vi "iBeam Laser Engine.vi"(0 "iBeam Laser Notifier":string, 11 "COM Port":string[](array[string])) -> ()   [LabVIEW 2016]
uses:
  Laser Controls/Laser Notifier Element.ctl
  Laser Controls/Laser Actions.ctl
  Laser Controls/Laser Settings.ctl
  Laser Controls/Laser Parameters.ctl
  Laser Controls/Laser Status.ctl
  <vilib>/Instr/_visa.llb/VISA Configure Serial Port (Instr).vi
panel:
  in  "Fine A":dbl
  in  "Fine B":dbl
  in  "Enable Fine":bool
  out "Channels":enum32{"Channel 1", "Channel 2"}(radio)
  in  "Get Status":bool
  in  "Get Power":bool
  out "Laser Status":string
  out "Power (uW)":string
  out "Startup Error":errorcluster
  in  "Quit":bool
  in  "Enable Ext":bool
  in  "Laser Power (mW)":dbl
  in  "Laser On/Off":bool
  out "Serial Number":string
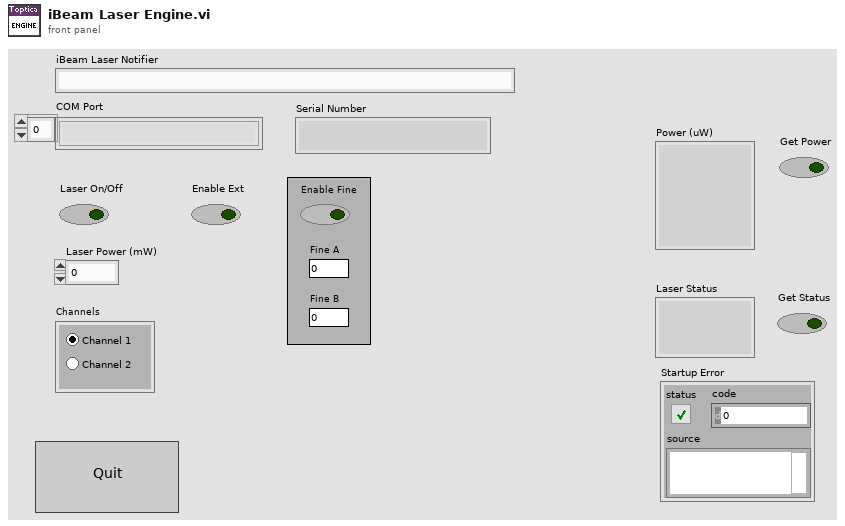
[diagram p1: front panel]
types:
  T1 = typedef "Laser Parameters.ctl" = enum16{"Wavelength (nm)", "Pulsing?", "Rep. Rate", "External Control", "Enable Fine", "Fine A", "Fine B", "Channel No."}
  T2 = typedef "Laser Notifier Element.ctl" = cluster{"Laser Action":T3, "Received?":bool, "Enabled (Interlock)?":bool, "Light Emission?":bool, "Power (mW)":dbl, "Settings":T4, "Status":T5, "Error":errorcluster}
  T3 = typedef "Laser Actions.ctl" = enum16{"Error Check", "Set On/Off", "Set Power", "Set Parameter", "Get Power", "Get Status", "Get Parameter", "Quit"}
  T4 = typedef "Laser Settings.ctl" = cluster{"Laser Parameters":T1, "Value":dbl}
  T5 = typedef "Laser Status.ctl" = enum16{"Warmup", "Ready", "Emission", "Tuning", "Error"}
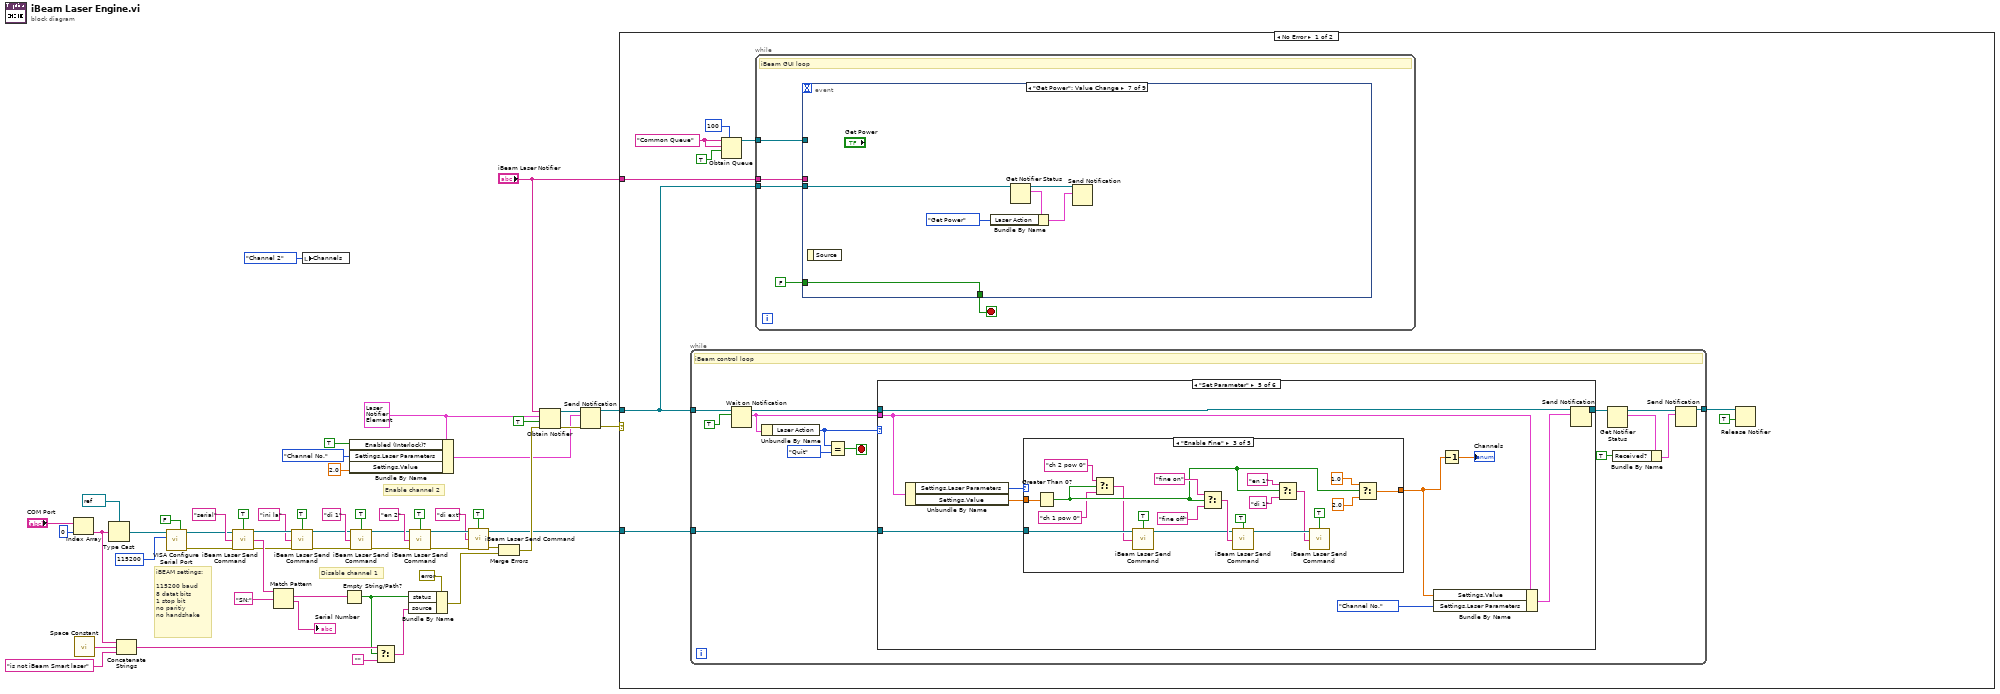
[diagram p0: block diagram]
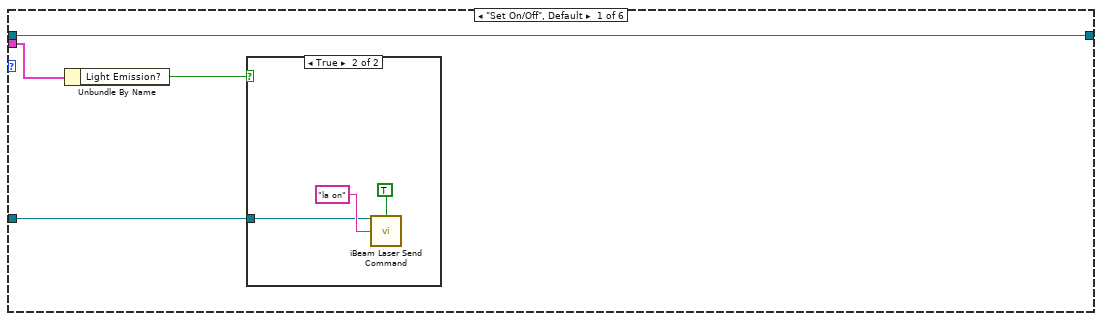
[diagram p2: hidden frame]
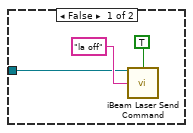
[diagram p3: hidden frame]
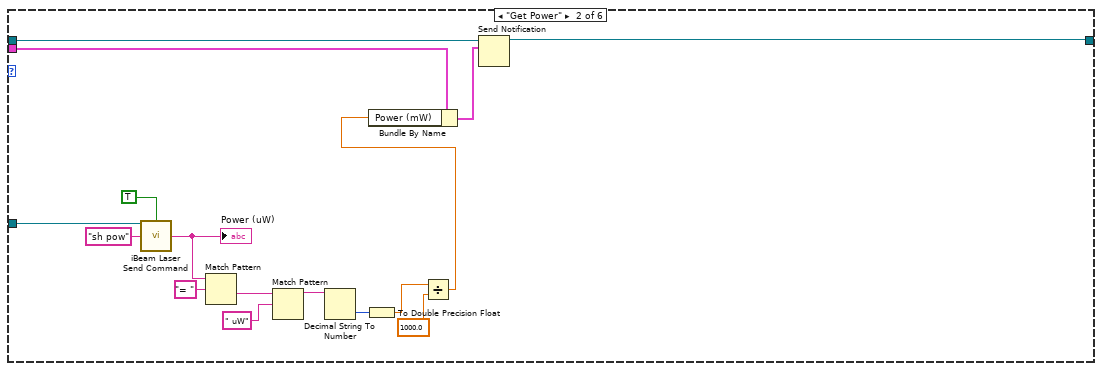
[diagram p4: hidden frame]
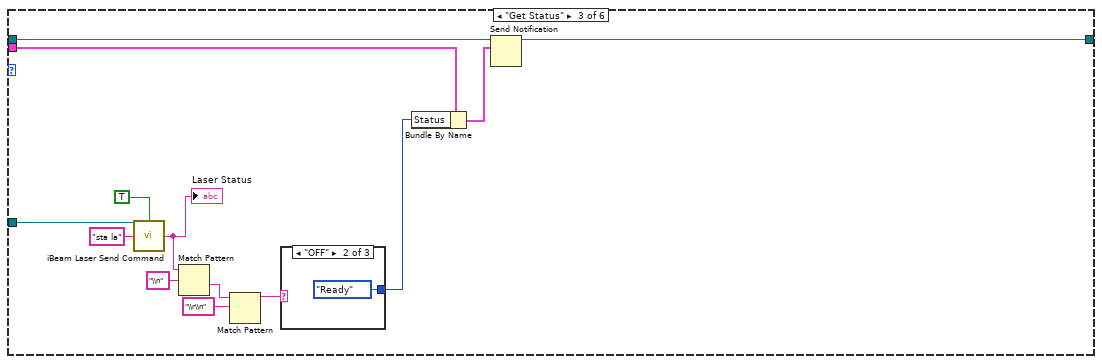
[diagram p5: hidden frame]
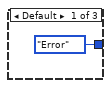
[diagram p6: hidden frame]
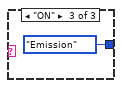
[diagram p7: hidden frame]
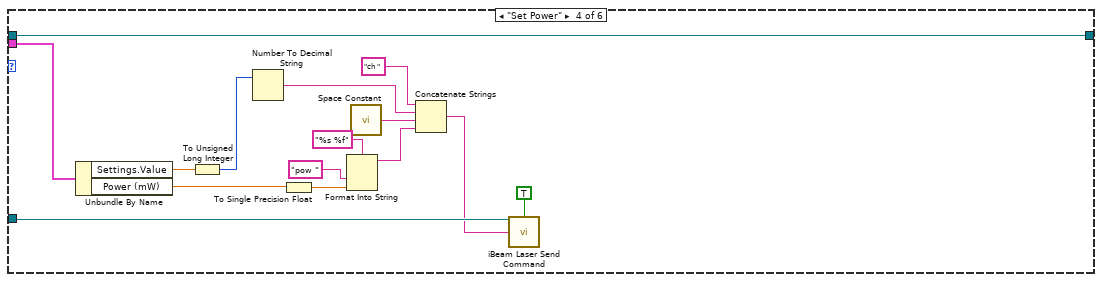
[diagram p8: hidden frame]
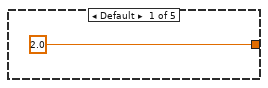
[diagram p9: hidden frame]
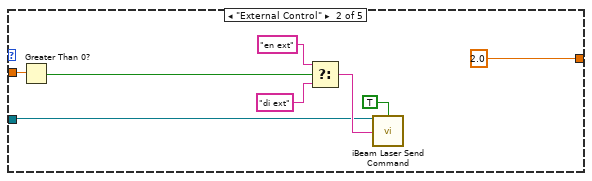
[diagram p10: hidden frame]
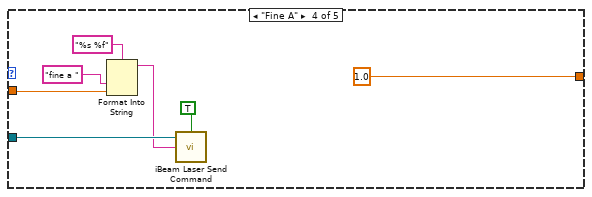
[diagram p11: hidden frame]
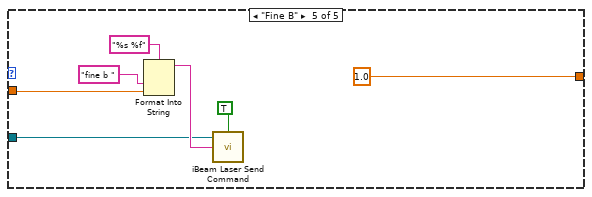
[diagram p12: hidden frame]
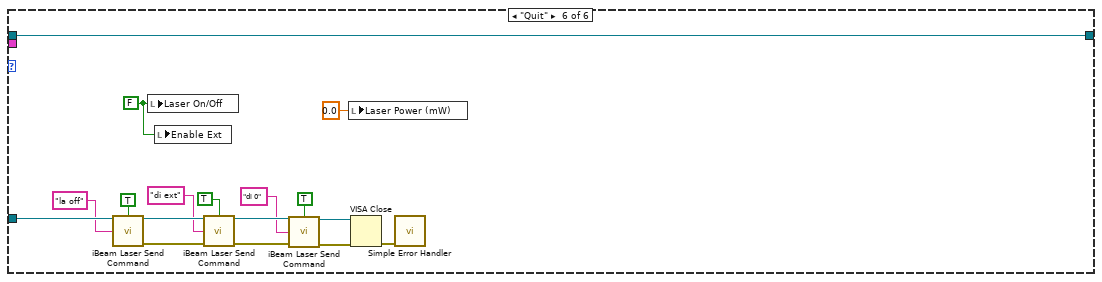
[diagram p13: hidden frame]
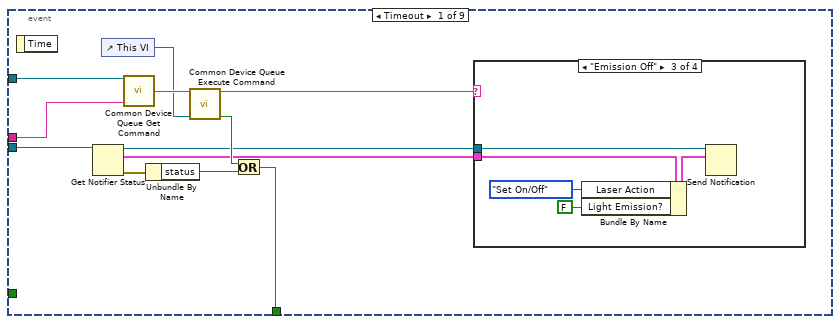
[diagram p14: hidden frame]
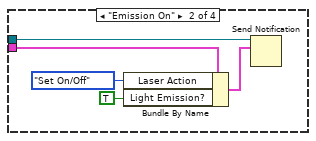
[diagram p16: hidden frame]
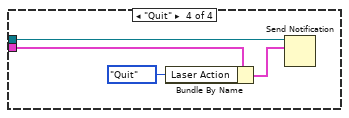
[diagram p17: hidden frame]
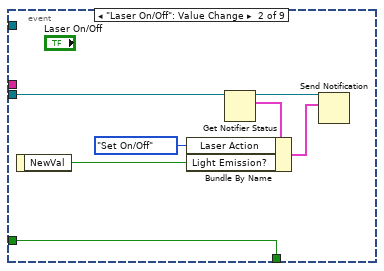
[diagram p18: hidden frame]
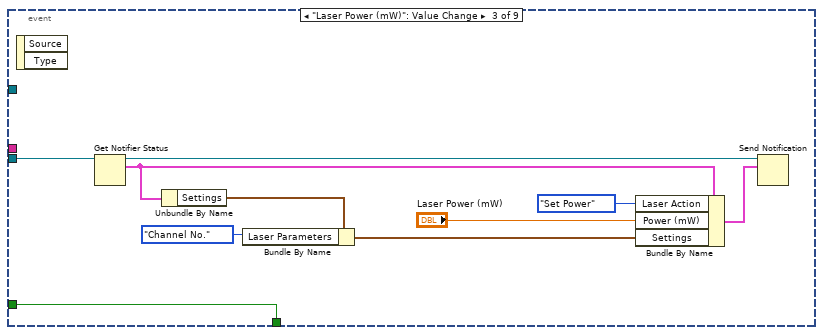
[diagram p19: hidden frame]
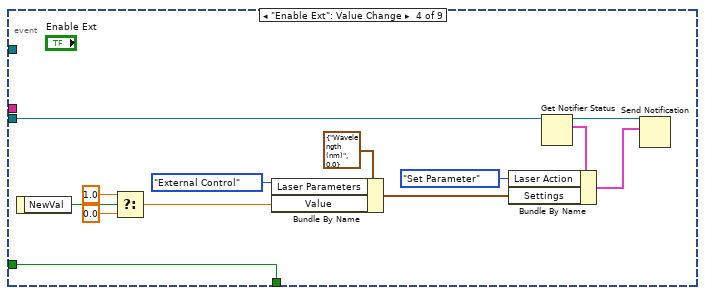
[diagram p20: hidden frame]
diagram:
  w17 = T2 {"Laser Action"=enum."Set On/Off", "Received?"=FALSE, "Enabled (Interlock)?"=FALSE, "Light Emission?"=FALSE, "Power (mW)"=0.0, "Settings"={"Laser Parameters"=enum."Wavelength (nm)", "Value"=0.0}, "Status"=enum."Error", "Error"={"status"=FALSE, "code"=0, "source"=""}} ("Laser Notifier Element")
  # "iBEAM settings:\n\n115200 baud\n8 datat bits\n1 stop bit\nno paritiy\nno handshake"
  # "Enable channel 2"
  # "Disable channel 1"
  n1 = Index Array(array="COM Port", index=0) -> (element=w47:string)
  n2 = call <vilib>:"Space Constant.vi"() -> ("String"=w46:string)
  n3 = Type Cast(type=refnum<visa-resource-name> refnum ("VISA resource name"), x=w47) -> (*(type *) &x=w6:refnum<visa-resource-name>)
  n4 = Concatenate Strings(w47, w46, "is not iBeam Smart laser" ("string")) -> (w43:string)
  n5 = call-poly "VISA Configure Serial Port"("VISA resource name"=w6, "Enable Termination\nChar (T)"=FALSE ("Enable Termination\nChar (T)"), "baud rate (9600)"=u32 115200 ("baud rate (115200)")) -> ("VISA resource name out"=w5:refnum<visa-resource-name>, "error out"=w4:errorcluster)  [unwired: 11 in]
  n6 = call "iBeam Laser Send Command.vi"("VISA Ref"=w5, "Wait for Reply?"=TRUE, "Command"="serial" ("command"), "Error In"=w4) -> ("VISA Ref Out"=w33:refnum<visa-resource-name>, "Response"=w50:string, "Error Out"=w32:errorcluster)  [unwired: 9 in]
  n7 = Match Pattern(string=w50, regular expression="SN:") -> (match substring=w44:string, after substring=→"Serial Number":string)  [unwired: 1 in, 2 out]
  n8 = call "iBeam Laser Send Command.vi"("VISA Ref"=w33, "Wait for Reply?"=TRUE, "Command"="ini la", "Error In"=w32) -> ("VISA Ref Out"=w25:refnum<visa-resource-name>, "Error Out"=w24:errorcluster)  [unwired: 9 in, 1 out]
  n9 = local write "Channels"(enum32{"Channel 1", "Channel 2"}."Channel 2" ("Channels")) -> ()
  n10 = Empty String/Path?(string/path=w44) -> (empty?=w40:bool)
  n11 = Bundle By Name(cluster=w17, "Enabled (Interlock)?"=TRUE, "Settings.Laser Parameters"=Laser_Parameters."Channel No.", "Settings.Value"=2.0) -> (w15:T2)
  n12 = call "iBeam Laser Send Command.vi"("VISA Ref"=w25, "Wait for Reply?"=TRUE, "Command"="di 1", "Error In"=w24) -> ("VISA Ref Out"=w22:refnum<visa-resource-name>, "Error Out"=w21:errorcluster)  [unwired: 9 in, 1 out]
  n13 = Select(t=w43, s=w40, f="") -> (s? t:f=w39:string)
  n14 = Bundle By Name(cluster=errorcluster {"status"=FALSE, "code"=0, "source"=""} ("error in"), "status"=w40, "source"=w39) -> (w38:errorcluster)
  n15 = call "iBeam Laser Send Command.vi"("VISA Ref"=w22, "Wait for Reply?"=TRUE, "Command"="en 2", "Error In"=w21) -> ("VISA Ref Out"=w14:refnum<visa-resource-name>, "Error Out"=w11:errorcluster)  [unwired: 9 in, 1 out]
  n16 = call "iBeam Laser Send Command.vi"("VISA Ref"=w14, "Wait for Reply?"=TRUE, "Command"="di ext", "Error In"=w11) -> ("VISA Ref Out"=w13:refnum<visa-resource-name>, "Error Out"=w10:errorcluster)  [unwired: 9 in, 1 out]
  n17 = Merge Errors(w10, w38) -> (w37:errorcluster)
  n18 = Obtain Notifier(name (unnamed)="iBeam Laser Notifier", notification data type=w17, create if not found? (T)=TRUE, error in (no error)=w37) -> (notifier out=w27:refnum<notifier>, error out=w36:errorcluster)  [unwired: 1 out]
  n19 = Send Notification(notification=w15, notifier=w27, error in (no error)=w36) -> (notifier out=w29:refnum<notifier>, error out=w35:errorcluster)
  n20 = case shown="No Error" w35 {
    selector: w35 -> [_ w310]
    tunnel: w29 -> [w63 w311]
    tunnel: w13 -> [w62 w309]
    tunnel: "iBeam Laser Notifier" -> [w56 _]
    frame No Error {
      w59 = "Common Queue" ("Unique Notifier Name")
      n21 = while {
        tunnel: w63 -> [w77]
        tunnel: w62 -> [w73]
        tunnel: [w65] -> w60
        stop <- w76 stop-if-true
        # "iBeam control loop"
        n22 = Wait on Notification(notifier=w77, ignore previous (F)=TRUE) -> (notifier out=w72:refnum<notifier>, notification=w74:T2)  [unwired: 2 in, 2 out]
        n23 = Unbundle By Name(w74) -> ("Laser Action"=w75:T3)
        n24 = Equal?(x=w75, y=Laser_Actions."Quit") -> (x = y?=w76:bool)
        n25 = case shown="\"Set Parameter\"" w75 {
          tunnel: w74 -> [w81 w92 w108 w134 w140 _]
          tunnel: w73 -> [w79 w103 w116 w129 w144 w204]
          tunnel: w72 -> [w78 w90 w105 w126 w138 w188]
          tunnel: [w78 w89 w104 w126 w139 w188] -> w70
          frame "Set On/Off", Default {
            n26 = Unbundle By Name(w81) -> ("Light Emission?"=w80:bool)
            n27 = case shown="True" w80 {
              tunnel: w79 -> [w82 w85]
              frame False {
                n28 = call "iBeam Laser Send Command.vi"("VISA Ref"=w82, "Wait for Reply?"=TRUE, "Command"="la off" ("command")) -> ()  [unwired: 10 in, 3 out]
              }
              frame True {
                n29 = call "iBeam Laser Send Command.vi"("VISA Ref"=w85, "Wait for Reply?"=TRUE, "Command"="la on" ("command")) -> ()  [unwired: 10 in, 3 out]
              }
            }
          }
          frame "Get Power" {
            n30 = call "iBeam Laser Send Command.vi"("VISA Ref"=w103, "Wait for Reply?"=TRUE, "Command"="sh pow") -> ("Response"=w100:string)  [unwired: 10 in, 2 out]
            "Power (uW)" <- w100
            n31 = Match Pattern(string=w100, regular expression="= ") -> (after substring=w98:string)  [unwired: 1 in, 3 out]
            n32 = Match Pattern(string=w98, regular expression=" uW") -> (before substring=w96:string)  [unwired: 1 in, 3 out]
            n33 = Decimal String To Number(string=w96) -> (number=w95:i32)  [unwired: 2 in, 1 out]
            n34 = To Double Precision Float(number=w95) -> (double precision float=w94:dbl)
            n35 = Divide(x=w94, y=1000.0) -> (x/y=w88:dbl)
            n36 = Bundle By Name(cluster=w92, "Power (mW)"=w88) -> (w91:T2)
            n37 = Send Notification(notification=w91, notifier=w90) -> (notifier out=w89:refnum<notifier>)  [unwired: 1 in, 1 out]
          }
          frame "Get Status" {
            n38 = call "iBeam Laser Send Command.vi"("VISA Ref"=w116, "Wait for Reply?"=TRUE, "Command"="sta la") -> ("Response"=w113:string)  [unwired: 10 in, 2 out]
            "Laser Status" <- w113
            n39 = Match Pattern(string=w113, regular expression="\\n") -> (after substring=w112:string)  [unwired: 1 in, 3 out]
            n40 = Match Pattern(string=w112, regular expression="\\r\\n") -> (before substring=w109:string)  [unwired: 1 in, 3 out]
            n41 = case shown="\"OFF\"" w109 {
              tunnel: [Laser_Status."Error" ("Status") Laser_Status."Ready" ("Status") Laser_Status."Emission" ("Status")] -> w107
              frame Default {
              }
              frame "OFF" {
              }
              frame "ON" {
              }
            }
            n42 = Bundle By Name(cluster=w108, "Status"=w107) -> (w106:T2)
            n43 = Send Notification(notification=w106, notifier=w105) -> (notifier out=w104:refnum<notifier>)  [unwired: 1 in, 1 out]
          }
          frame "Set Power" {
            n44 = Unbundle By Name(w134) -> ("Settings.Value"=w123:dbl, "Power (mW)"=w125:dbl)
            n45 = To Unsigned Long Integer(number=w123) -> (unsigned 32bit integer=w121:u32)
            n46 = Number To Decimal String(number=w121) -> (decimal integer string=w120:string)  [unwired: 1 in]
            n47 = To Single Precision Float(number=w125) -> (single precision float=w124:sgl)
            n48 = Format Into String(format string="%s %f", "pow " ("string"), w124) -> (resulting string=w130:string)  [unwired: 2 in, 1 out]
            n49 = call <vilib>:"Space Constant.vi"() -> ("String"=w131:string)
            n50 = Concatenate Strings("ch " ("string"), w120, w131, w130) -> (w128:string)
            n51 = call "iBeam Laser Send Command.vi"("VISA Ref"=w129, "Wait for Reply?"=TRUE, "Command"=w128) -> ()  [unwired: 10 in, 3 out]
          }
          frame "Set Parameter" {
            n52 = Unbundle By Name(w140) -> ("Settings.Laser Parameters"=w143:T1, "Settings.Value"=w142:dbl)
            n53 = case shown="\"Enable Fine\"" w143 {
              tunnel: w144 -> [_ w146 w159 w176 w182]
              tunnel: w142 -> [_ w152 w169 w178 w183]
              tunnel: [2.0 ("f") 2.0 ("f") w161 1.0 ("f") 1.0 ("f")] -> w136
              frame Default {
              }
              frame "External Control" {
                n54 = Greater Than 0?(x=w152) -> (x > 0?=w148:bool)
                n55 = Select(t="en ext" ("Command"), s=w148, f="di ext" ("Command")) -> (s? t:f=w149:string)
                n56 = call "iBeam Laser Send Command.vi"("VISA Ref"=w146, "Wait for Reply?"=TRUE, "Command"=w149) -> ()  [unwired: 10 in, 3 out]
              }
              frame "Enable Fine" {
                n57 = Greater Than 0?(x=w169) -> (x > 0?=w157:bool)
                n58 = Select(t="ch 2 pow 0" ("Command"), s=w157, f="ch 1 pow 0") -> (s? t:f=w154:string)
                n59 = call "iBeam Laser Send Command.vi"("VISA Ref"=w159, "Wait for Reply?"=TRUE, "Command"=w154) -> ("VISA Ref Out"=w158:refnum<visa-resource-name>)  [unwired: 10 in, 2 out]
                n60 = Select(t="fine on" ("Command"), s=w157, f="fine off" ("Command")) -> (s? t:f=w173:string)
                n61 = call "iBeam Laser Send Command.vi"("VISA Ref"=w158, "Wait for Reply?"=TRUE, "Command"=w173) -> ("VISA Ref Out"=w167:refnum<visa-resource-name>)  [unwired: 10 in, 2 out]
                n62 = Select(t="en 1" ("Command"), s=w157, f="di 1") -> (s? t:f=w164:string)
                n63 = call "iBeam Laser Send Command.vi"("VISA Ref"=w167, "Wait for Reply?"=TRUE, "Command"=w164) -> ()  [unwired: 10 in, 3 out]
                n64 = Select(t=1.0, s=w157, f=2.0) -> (s? t:f=w161:dbl)
              }
              frame "Fine A" {
                n65 = Format Into String(format string="%s %f", "fine a " ("string"), w178) -> (resulting string=w175:string)  [unwired: 2 in, 1 out]
                n66 = call "iBeam Laser Send Command.vi"("VISA Ref"=w176, "Wait for Reply?"=TRUE, "Command"=w175) -> ()  [unwired: 10 in, 3 out]
              }
              frame "Fine B" {
                n67 = Format Into String(format string="%s %f", "fine b " ("string"), w183) -> (resulting string=w187:string)  [unwired: 2 in, 1 out]
                n68 = call "iBeam Laser Send Command.vi"("VISA Ref"=w182, "Wait for Reply?"=TRUE, "Command"=w187) -> ()  [unwired: 10 in, 3 out]
              }
            }
            n69 = Bundle By Name(cluster=w140, "Settings.Value"=w136, "Settings.Laser Parameters"=Laser_Parameters."Channel No." ("Laser Parameters")) -> (w137:T2)
            n70 = Decrement(x=w136) -> (x-1=→"Channels":dbl)
            n71 = Send Notification(notification=w137, notifier=w138) -> (notifier out=w139:refnum<notifier>)  [unwired: 1 in, 1 out]
          }
          frame "Quit" {
            w190 = FALSE ("Laser On/Off")
            n72 = call "iBeam Laser Send Command.vi"("VISA Ref"=w204, "Wait for Reply?"=TRUE, "Command"="la off") -> ("VISA Ref Out"=w202:refnum<visa-resource-name>, "Error Out"=w201:errorcluster)  [unwired: 10 in, 1 out]
            n73 = local write "Laser On/Off"(w190) -> ()
            n74 = local write "Enable Ext"(w190) -> ()
            n75 = call "iBeam Laser Send Command.vi"("VISA Ref"=w202, "Wait for Reply?"=TRUE, "Command"="di ext", "Error In"=w201) -> ("VISA Ref Out"=w196:refnum<visa-resource-name>, "Error Out"=w195:errorcluster)  [unwired: 9 in, 1 out]
            n76 = call "iBeam Laser Send Command.vi"("VISA Ref"=w196, "Wait for Reply?"=TRUE, "Command"="di 0", "Error In"=w195) -> ("VISA Ref Out"=w194:refnum<visa-resource-name>, "Error Out"=w193:errorcluster)  [unwired: 9 in, 1 out]
            n77 = local write "Laser Power (mW)"(sgl 0.0 ("Laser Power (mW)")) -> ()
            n78 = VISA Close(VISA resource name=w194, error in (no error)=w193) -> (error out=w199:errorcluster)
            n79 = call <vilib>:"Simple Error Handler.vi"("error in (no error)"=w199) -> ()  [unwired: 4 in, 5 out]
          }
        }
        n80 = Get Notifier Status(notifier=w70) -> (notifier out=w67:refnum<notifier>, current notification=w69:T2)  [unwired: 1 in, 3 out]
        n81 = Bundle By Name(cluster=w69, "Received?"=TRUE) -> (w66:T2)
        n82 = Send Notification(notification=w66, notifier=w67) -> (notifier out=w65:refnum<notifier>)  [unwired: 1 in, 1 out]
      }
      n83 = Obtain Queue(max queue size (-1, unlimited)=100, name (unnamed)=w59, element data type=w59, create if not found? (T)=TRUE) -> (queue out=w55:refnum<queue>)  [unwired: 1 in, 2 out]
      n84 = while {
        tunnel: w63 -> [w209]
        tunnel: w56 -> [w206]
        tunnel: w55 -> [w205]
        stop <- w207 stop-if-true
        # "iBeam GUI loop"
        n85 = event shown="[6] \"Get Power\": Value Change" {
          selector: _ -> [_ _ _ _ _ _ _ _ _]
          dyn-events: _ -> [_ _ _ _ _ _ _ _ _]
          timeout: _ -> [_ _ _ _ _ _ _ _ _]
          tunnel: w209 -> [w216 w242 w252 w265 w266 w284 w293 w298 w306]
          tunnel: FALSE ("stop") -> [_ w237 w249 w261 _ _ w291 w297 _]
          tunnel: [w212 w237 w249 w261 _ _ w291 w297 w308] -> w207
          tunnel: w206 -> [w220 _ _ _ _ _ _ _ _]
          tunnel: w205 -> [w221 _ _ _ _ _ _ _ _]
          event Timeout {
            n86 = event-data() -> ()  [unwired: 1 in, 1 out]
            n87 = Get Notifier Status(notifier=w216) -> (notifier out=w211:refnum<notifier>, current notification=w210:T2, error out=w215:errorcluster)  [unwired: 1 in, 2 out]
            n88 = control-ref of="This VI"() -> (w218:refnum<vi>)
            n89 = call "Common Device Queue Get Command.vi"("Common Queue"=w221, "Notifier Name"=w220) -> ("Command"=w219:string)  [unwired: 12 in, 1 out]
            n90 = Unbundle By Name(w215) -> ("status"=w213:bool)
            n91 = call "Common Device Queue Execute Command.vi"("Common Command"=w219, "VI Refnum"=w218) -> ("Common Command"=w217:string, "Quit?"=w214:bool)  [unwired: 12 in]
            n92 = Or(x=w214, y=w213) -> (x .or. y?=w212:bool)
            n93 = case shown="\"Emission Off\"" w217 {
              tunnel: w211 -> [_ w226 w229 w234]
              tunnel: w210 -> [_ w225 w228 w233]
              frame Default {
              }
              frame "Emission On" {
                n94 = Bundle By Name(cluster=w225, "Laser Action"=Laser_Actions."Set On/Off", "Light Emission?"=TRUE) -> (w224:T2)
                n95 = Send Notification(notification=w224, notifier=w226) -> ()  [unwired: 1 in, 2 out]
              }
              frame "Emission Off" {
                n96 = Bundle By Name(cluster=w228, "Laser Action"=Laser_Actions."Set On/Off", "Light Emission?"=FALSE) -> (w230:T2)
                n97 = Send Notification(notification=w230, notifier=w229) -> ()  [unwired: 1 in, 2 out]
              }
              frame "Quit" {
                n98 = Bundle By Name(cluster=w233, "Laser Action"=Laser_Actions."Quit") -> (w235:T2)
                n99 = Send Notification(notification=w235, notifier=w234) -> ()  [unwired: 1 in, 2 out]
              }
            }
          }
          event "Laser On/Off": Value Change {
            n100 = event-data() -> ("NewVal"=w240:bool)  [unwired: 1 in]
            n101 = Get Notifier Status(notifier=w242) -> (notifier out=w241:refnum<notifier>, current notification=w238:T2)  [unwired: 1 in, 3 out]
            n102 = Bundle By Name(cluster=w238, "Laser Action"=Laser_Actions."Set On/Off", "Light Emission?"=w240) -> (w239:T2)
            n103 = Send Notification(notification=w239, notifier=w241) -> ()  [unwired: 1 in, 2 out]
          }
          event "Laser Power (mW)": Value Change {
            n104 = event-data() -> ()  [unwired: 1 in, 2 out]
            n105 = Get Notifier Status(notifier=w252) -> (notifier out=w251:refnum<notifier>, current notification=w244:T2)  [unwired: 1 in, 3 out]
            n106 = Unbundle By Name(w244) -> ("Settings"=w243:T4)
            n107 = Bundle By Name(cluster=w243, "Laser Parameters"=Laser_Parameters."Channel No.") -> (w245:T4)
            n108 = Bundle By Name(cluster=w244, "Laser Action"=Laser_Actions."Set Power", "Power (mW)"="Laser Power (mW)", "Settings"=w245) -> (w250:T2)
            n109 = Send Notification(notification=w250, notifier=w251) -> ()  [unwired: 1 in, 2 out]
          }
          event "Enable Ext": Value Change {
            n110 = event-data() -> ("NewVal"=w256:bool)  [unwired: 1 in]
            n111 = Select(t=1.0, s=w256, f=0.0) -> (s? t:f=w253:dbl)
            n112 = Bundle By Name(cluster=T4 {"Laser Parameters"=enum."Wavelength (nm)", "Value"=0.0} ("Settings"), "Laser Parameters"=Laser_Parameters."External Control", "Value"=w253) -> (w258:T4)
            n113 = Get Notifier Status(notifier=w265) -> (notifier out=w263:refnum<notifier>, current notification=w264:T2)  [unwired: 1 in, 3 out]
            n114 = Bundle By Name(cluster=w264, "Laser Action"=Laser_Actions."Set Parameter", "Settings"=w258) -> (w262:T2)
            n115 = Send Notification(notification=w262, notifier=w263) -> ()  [unwired: 1 in, 2 out]
          }
          event "Enable Fine": Value Change {
            n116 = event-data() -> ("NewVal"=w268:bool)  [unwired: 1 in]
            n117 = Select(t=1.0, s=w268, f=0.0) -> (s? t:f=w269:dbl)
            n118 = Bundle By Name(cluster=T4 {"Laser Parameters"=enum."Wavelength (nm)", "Value"=0.0} ("Settings"), "Laser Parameters"=Laser_Parameters."Enable Fine", "Value"=w269) -> (w273:T4)
            n119 = Get Notifier Status(notifier=w266) -> (notifier out=w276:refnum<notifier>, current notification=w277:T2)  [unwired: 1 in, 3 out]
            n120 = Bundle By Name(cluster=w277, "Laser Action"=Laser_Actions."Set Parameter", "Settings"=w273) -> (w275:T2)
            n121 = Send Notification(notification=w275, notifier=w276) -> ()  [unwired: 1 in, 2 out]
          }
          event "Fine B", "Fine A": Value Change {
            n122 = event-data() -> ("CtlRef"=w286:refnum<vi>)  [unwired: 1 in]
            n123 = Get Notifier Status(notifier=w284) -> (notifier out=w280:refnum<notifier>, current notification=w283:T2)  [unwired: 1 in, 3 out]
            n124 = property class="DigNum (strict)"(reference=w286) -> ("Label.Text"=w285:string)  [unwired: 1 in, 2 out]
            n125 = case shown="\"Fine A\", Default" w285 {
              tunnel: ["Fine A" "Fine B"] -> w281
              tunnel: [Laser_Parameters."Fine A" ("Settings.Laser Parameters") Laser_Parameters."Fine B" ("Settings.Laser Parameters")] -> w282
              frame "Fine A", Default {
              }
              frame "Fine B" {
              }
            }
            n126 = Bundle By Name(cluster=w283, "Settings.Value"=w281, "Settings.Laser Parameters"=w282, "Laser Action"=Laser_Actions."Set Parameter") -> (w279:T2)
            n127 = Send Notification(notification=w279, notifier=w280) -> ()  [unwired: 1 in, 2 out]
          }
          event "Get Power": Value Change {
            n128 = event-data() -> ()  [unwired: 1 in, 1 out]
            n129 = Get Notifier Status(notifier=w293) -> (notifier out=w296:refnum<notifier>, current notification=w295:T2)  [unwired: 1 in, 3 out]
            n130 = Bundle By Name(cluster=w295, "Laser Action"=Laser_Actions."Get Power") -> (w292:T2)
            n131 = Send Notification(notification=w292, notifier=w296) -> ()  [unwired: 1 in, 2 out]
          }
          event "Get Status": Value Change {
            n132 = event-data() -> ()  [unwired: 1 in, 1 out]
            n133 = Get Notifier Status(notifier=w298) -> (notifier out=w302:refnum<notifier>, current notification=w301:T2)  [unwired: 1 in, 3 out]
            n134 = Bundle By Name(cluster=w301, "Laser Action"=Laser_Actions."Get Status") -> (w299:T2)
            n135 = Send Notification(notification=w299, notifier=w302) -> ()  [unwired: 1 in, 2 out]
          }
          event "Quit": Value Change {
            n136 = event-data() -> ("NewVal"=w308:bool)  [unwired: 1 in]
            n137 = Get Notifier Status(notifier=w306) -> (notifier out=w307:refnum<notifier>, current notification=w305:T2)  [unwired: 1 in, 3 out]
            n138 = Bundle By Name(cluster=w305, "Laser Action"=Laser_Actions."Quit") -> (w304:T2)
            n139 = Send Notification(notification=w304, notifier=w307) -> ()  [unwired: 1 in, 2 out]
          }
        }
      }
      n140 = Release Notifier(notifier=w60, force destroy? (F)=TRUE) -> ()  [unwired: 1 in, 3 out]
    }
    frame Error {
      n141 = VISA Close(VISA resource name=w309, error in (no error)=w310) -> (error out=w313:errorcluster)
      n142 = Release Notifier(notifier=w311, force destroy? (F)=TRUE, error in (no error)=w313) -> (error out=→"Startup Error":errorcluster)  [unwired: 2 out]
    }
  }
